vi "midiOutPlayer.Launch.vi"(8 "error in":errorcluster, 11 "midiPlayer in":refnum<class "midiPlayer.lvclass">) -> (0 "error out":errorcluster, 3 "midiPlayer out":refnum<class "midiPlayer.lvclass">)   [LabVIEW 2020, in "midiPlayer.lvclass"]
uses:
  midiPlayer.lvclass
  midiPlayer.lvclass/midiPlayer.ctl
  midiOutPlayer.Core.vi
  midi-file-events/midi-file-events.lvclass
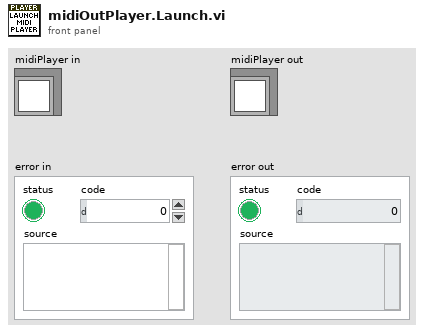
[diagram p1: front panel]
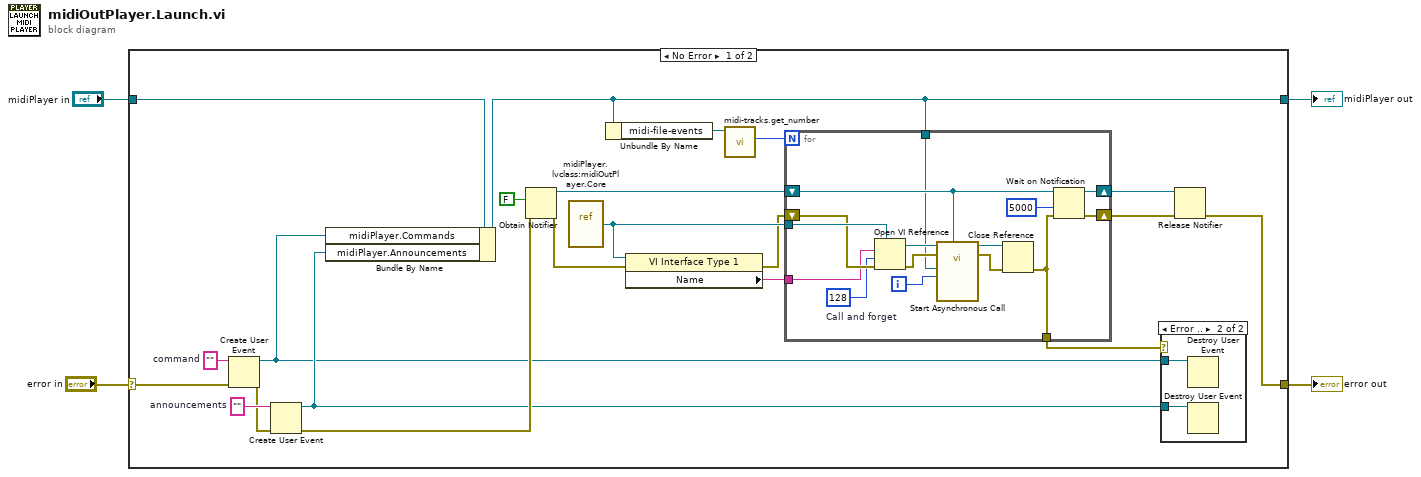
[diagram p0: block diagram]
diagram:
  n1 = case shown="No Error" "error in" {
    selector: "error in" -> [w19 w44]
    tunnel: [w9 w44] -> w3
    tunnel: "midiPlayer in" -> [w8 w43]
    tunnel: [w6 w43] -> w1
    frame No Error {
      w18 = ""  # announcements
      w25 = ""  # command
      n2 = Create User Event(user event datatype=w25, error in=w19) -> (user event=w10:refnum<user-event>, error out=w17:errorcluster)
      n3 = Create User Event(user event datatype=w18, error in=w17) -> (user event=w11:refnum<user-event>, error out=w16:errorcluster)
      n4 = Bundle By Name(cluster=w8, "midiPlayer.Commands"=w10, "midiPlayer.Announcements"=w11) -> (w6:refnum<class "midiPlayer.lvclass">)
      n5 = Obtain Notifier(notification data type=FALSE, error in (no error)=w16) -> (notifier out=w15:refnum<notifier>, error out=w20:errorcluster)  [unwired: 2 in, 1 out]
      n6 = vi-ref "midiPlayer.lvclass:midiOutPlayer.Core.vi"() -> (w23:refnum<vi>)
      n7 = Unbundle By Name(w6) -> ("midi-file-events"=w7:refnum<class "midi-file-events.lvclass">)
      n8 = property class="VI Interface Type 1"(reference=w23, error in=w20) -> (error out=w22:errorcluster, "Name"=w21:string)  [unwired: 1 out]
      n9 = call "midi-tracks.get_number.vi"("midi-file-events in"=w7) -> ("Numer of Tracks"=w5:i32)  [unwired: 8 in, 2 out]
      n10 = for {
        N: w5 -> [_]
        tunnel: w23 -> [w38]
        tunnel: w21 -> [w36]
        tunnel: [w31] -> w14
        tunnel: w6 -> [w27]
        shift-right: [w29] -> w12
        shift-left: w22 -> [w37]
        shift-right: [w30] -> w13
        shift-left: w15 -> [w32]
        i -> [w26]
        w35 = 128  # Call and forget
        n11 = Open VI Reference(type specifier VI Refnum (for type only)=w38, vi path=w36, options=w35, error in (no error)=w37) -> (vi reference=w39:refnum<vi>, error out=w40:errorcluster)  [unwired: 2 in]
        n12 = call-by-ref "Start Asynchronous Call"(reference=w39, error in=w40, "notifier out"=w32, "Track Number"=w26, "midiPlayer"=w27) -> (reference out=w34:refnum<vi>, error out=w33:errorcluster)  [unwired: 9 in]
        n13 = Close Reference(reference=w34, error in (no error)=w33) -> (error out=w31:errorcluster)
        n14 = Wait on Notification(notifier=w32, timeout in ms (-1)=5000, error in (no error)=w31) -> (notifier out=w30:refnum<notifier>, error out=w29:errorcluster)  [unwired: 1 in, 2 out]
      }
      n15 = case shown="Error .." w14 {
        tunnel: w10 -> [_ w42]
        tunnel: w11 -> [_ w41]
        frame No Error {
        }
        frame Error {
          n16 = Destroy User Event(user event=w42) -> ()  [unwired: 1 in, 1 out]
          n17 = Destroy User Event(user event=w41) -> ()  [unwired: 1 in, 1 out]
        }
      }
      n18 = Release Notifier(notifier=w13, error in (no error)=w12) -> (error out=w9:errorcluster)  [unwired: 1 in, 2 out]
    }
    frame Error {
    }
  }
  "error out" <- w3
  "midiPlayer out" <- w1
